vi "RemoteVI Dirty Rects.vi"(9 "tile size":i32=64, 10 "current":u32[][](array[numeric]), 11 "previous":u32[][](array[numeric])) -> (3 "rects":cluster{"x":i32, "y":i32, "w":i32, "h":i32}[](array[cluster]))   [LabVIEW 2020, in "RemoteVI.lvlib"]
doc: "Compares two panel captures (2D U32 pixmaps [row, column], 0x00RRGGBB) in a grid of tile size x tile size tiles and returns the rectangles that changed. The dirty tiles of each tile row are merged into ONE rectangle from the first dirty tile's left edge to the last dirty tile's right edge (tiles are clipped at the panel edges; RemoteVI Dirty Band.vi); rows without a dirty tile give no rectangle. A tile row whose whole band is unchanged is skipped with a single comparison. If previous is empty or its dimensions differ from current, the result is one rectangle covering the whole current panel. A band or tile is unchanged when every pixel is equal (Equal? then And Array Elements). A tile size below 1 is treated as 1. Pure and reentrant: no error terminals because nothing here can fail. Mirrors dirtyRects() in tools/lib/rects.mjs."
uses:
  RemoteVI.lvlib
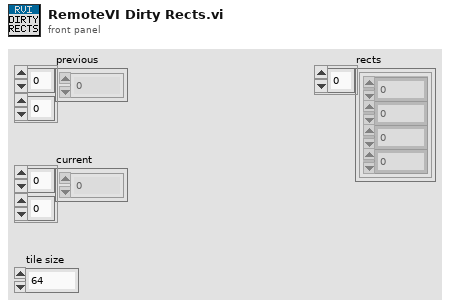
[diagram p1: front panel]
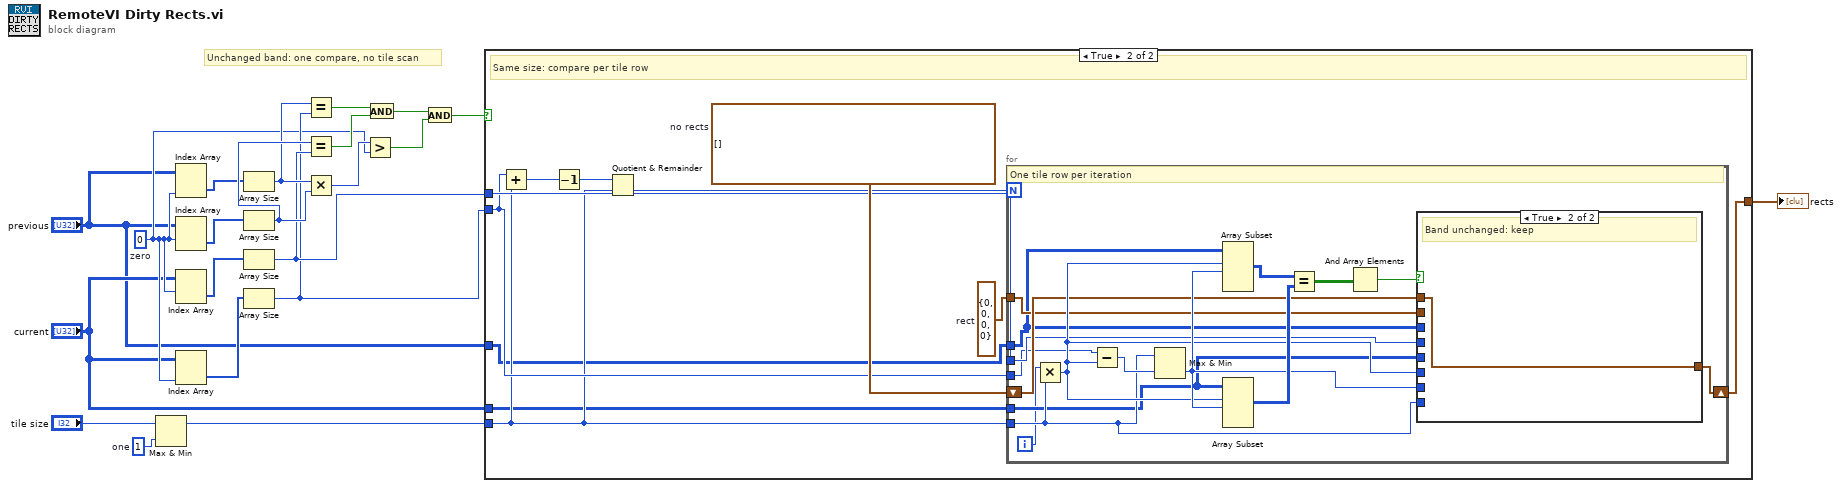
[diagram p0: block diagram]
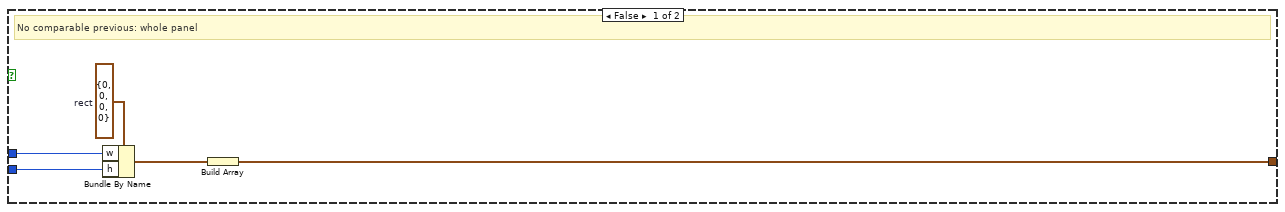
[diagram p2: hidden frame]
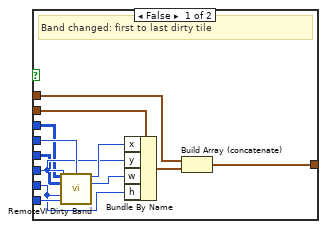
[diagram p3: hidden frame]
diagram:
  w5 = 0  # zero
  w4 = 1  # one
  # "Unchanged band: one compare, no tile scan"
  n1 = Max & Min(x="tile size", y=w4) -> (max(x,y)=w6:i32)  [unwired: 1 out]
  n2 = Index Array(array="previous", index (col)=w5) -> (element=w11:u32[])  [unwired: 1 in]
  n3 = Index Array(array="previous", index (row)=w5) -> (element=w13:u32[])  [unwired: 1 in]
  n4 = Index Array(array="current", index (row)=w5) -> (element=w9:u32[])  [unwired: 1 in]
  n5 = Index Array(array="current", index (col)=w5) -> (element=w7:u32[])  [unwired: 1 in]
  n6 = Array Size(array=w11) -> (size(s)=w12:i32)
  n7 = Array Size(array=w13) -> (size(s)=w14:i32)
  n8 = Array Size(array=w9) -> (size(s)=w10:i32)
  n9 = Array Size(array=w7) -> (size(s)=w8:i32)
  n10 = Equal?(x=w12, y=w8) -> (x = y?=w15:bool)
  n11 = Equal?(x=w14, y=w10) -> (x = y?=w16:bool)
  n12 = Multiply(x=w12, y=w14) -> (x*y=w17:i32)
  n13 = Greater?(x=w17, y=w5) -> (0:w18:bool)
  n14 = And(x=w15, y=w16) -> (x .and. y?=w19:bool)
  n15 = And(x=w19, y=w18) -> (x .and. y?=w20:bool)
  n16 = case shown="True" w20 {
    tunnel: "previous" -> [_ w27]
    tunnel: "current" -> [_ w28]
    tunnel: w6 -> [_ w29]
    tunnel: w8 -> [w22 w30]
    tunnel: w10 -> [w23 w31]
    tunnel: [w26 w37] -> w21
    frame False {
      w24 = cluster{"x":i32, "y":i32, "w":i32, "h":i32} {"x"=0, "y"=0, "w"=0, "h"=0}  # rect
      # "No comparable previous: whole panel"
      n17 = Bundle By Name(cluster=w24, "w"=w23, "h"=w22) -> (w25:cluster{"x":i32, "y":i32, "w":i32, "h":i32})
      n18 = Build Array(w25) -> (w26:cluster{"x":i32, "y":i32, "w":i32, "h":i32}[])
    }
    frame True {
      w36 = cluster{"x":i32, "y":i32, "w":i32, "h":i32} {"x"=0, "y"=0, "w"=0, "h"=0}  # rect
      w35 = cluster{"x":i32, "y":i32, "w":i32, "h":i32}[] []  # no rects
      # "Same size: compare per tile row"
      n19 = Add(x=w30, y=w29) -> (x+y=w32:i32)
      n20 = Decrement(x=w32) -> (x-1=w33:i32)
      n21 = Quotient & Remainder(x=w33, y=w29) -> (floor(x/y)=w34:i32)  [unwired: 1 out]
      n22 = for {
        N: w34 -> [_]
        tunnel: w36 -> [w44]
        shift-right: [w46] -> w37
        shift-left: w35 -> [w45]
        tunnel: w27 -> [w39]
        tunnel: w28 -> [w40]
        tunnel: w29 -> [w41]
        tunnel: w30 -> [w42]
        tunnel: w31 -> [w43]
        i -> [w38]
        # "One tile row per iteration"
        n23 = Multiply(x=w38, y=w41) -> (x*y=w47:i32)
        n24 = Subtract(x=w42, y=w47) -> (x-y=w48:i32)
        n25 = Max & Min(x=w41, y=w48) -> (min(x,y)=w49:i32)  [unwired: 1 out]
        n26 = Array Subset(array=w39, index (row)=w47, length (row)=w49) -> (w50:u32[][])  [unwired: 2 in]
        n27 = Array Subset(array=w40, index (row)=w47, length (row)=w49) -> (w51:u32[][])  [unwired: 2 in]
        n28 = Equal?(x=w50, y=w51) -> (x = y?=w52:bool[][])
        n29 = And Array Elements(Boolean array=w52) -> (logical AND=w53:bool)
        n30 = case shown="True" w53 {
          tunnel: w45 -> [w54 w66]
          tunnel: w44 -> [w61 _]
          tunnel: w39 -> [w55 _]
          tunnel: w40 -> [w56 _]
          tunnel: [w65 w66] -> w46
          tunnel: w41 -> [w59 _]
          tunnel: w47 -> [w57 _]
          tunnel: w43 -> [w60 _]
          tunnel: w49 -> [w58 _]
          frame False {
            # "Band changed: first to last dirty tile"
            n31 = call "RemoteVI Dirty Band.vi"("previous"=w55, "tile size"=w59, "width"=w60, "current"=w56, "y"=w57, "h"=w58) -> ("x"=w62:i32, "w"=w63:i32)  [unwired: 8 in]
            n32 = Bundle By Name(cluster=w61, "x"=w62, "y"=w57, "w"=w63, "h"=w58) -> (w64:cluster{"x":i32, "y":i32, "w":i32, "h":i32})
            n33 = Build Array (concatenate)(w54, w64) -> (w65:cluster{"x":i32, "y":i32, "w":i32, "h":i32}[])
          }
          frame True {
            # "Band unchanged: keep"
          }
        }
      }
    }
  }
  "rects" <- w21
